vi "Test_sqlite.vi"() -> ()   [LabVIEW 2020]
uses:
  <vilib>/Viviota/shared/ORM.lvlibp/TypeMap/TypeMap.lvclass
  DbConnections/SqliteConnection/DBC.lvclass
  C:/Program Files/National Instruments/LabVIEW 2020/vi.lib/Viviota/shared/ORM.lvlibp/DbConnection/DbConnection.lvclass
  <vilib>/Viviota/shared/ORM_ADONet.lvlibp/ADOMapper/ADOMapper.lvclass
  C:/Program Files/National Instruments/LabVIEW 2020/vi.lib/Viviota/shared/ORM.lvlibp/SqlMapper/SqlMapper.lvclass
  <vilib>/Viviota/shared/ORM_lib.lvlibp/ObjectRow/ObjectLUT.lvclass
  <vilib>/numeric/Random Number (Range) I64.vi
  <vilib>/numeric/Random Number (Range) DBL.vi
  f3693442-7653-4e44-a421-498bef5f0c13.vi
  <vilib>/Analysis/baseanly.llb/Mean (DBL).vi
  <vilib>/numeric/sub_Random U32.vi
  <vilib>/JDP Science/JSONtext/Variant to JSON Text.vi
  <vilib>/Viviota/shared/ORM_lib.lvlibp/ObjectRow/Write LUT.vi
  <vilib>/Viviota/shared/ORM.lvlibp/DbConnection/Write SupportTX.vi
  <vilib>/Viviota/shared/ORM.lvlibp/SqlMapper/Write DbConnection.vi
  <vilib>/Viviota/shared/ORM.lvlibp/TypeMap/Write Table Name.vi
  <vilib>/Viviota/shared/ORM.lvlibp/TypeMap/Write Autokey.vi
  <vilib>/Viviota/shared/ORM.lvlibp/TypeMap/Write ExcludeIDFromQueryParam.vi
  <vilib>/Viviota/shared/ORM_lib.lvlibp/ObjectRow/Read LUT.vi
  <vilib>/JDP Science/JSONtext/LVClass Serializer/JSONtext LVClass Serializer.lvclass
  <vilib>/Analysis/NI_AALBase.lvlib
panel:
  out "error out":errorcluster
  out "mean 3":dbl format="%0.6f"
  out "mean 2":dbl format="%0.6f"
  out "mean":dbl format="%0.6f"
  out "x-y":dbl[](array[numeric])
  out "Array 2":dbl[](array[numeric])
  out "Array":dbl[](array[numeric])
  out "LUT 2":variant[](array[variant])
  out "LUT":variant[](array[variant])
  out "id":i32[](array[numeric])
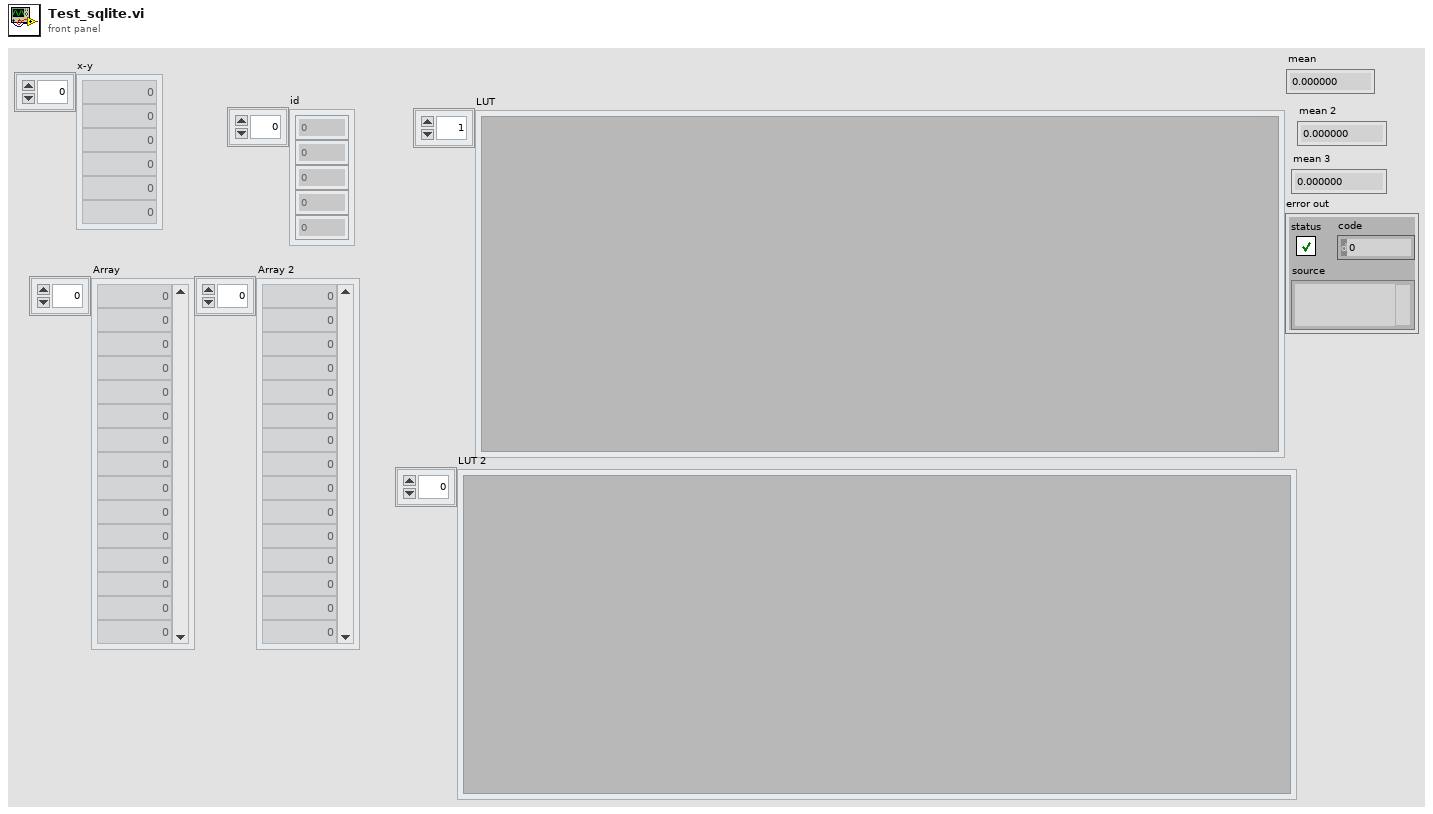
[diagram p1: front panel]
types:
  T1 = cluster{"Text":string, "Integer":i32, "dbl":dbl, "timestamp":timestamp}
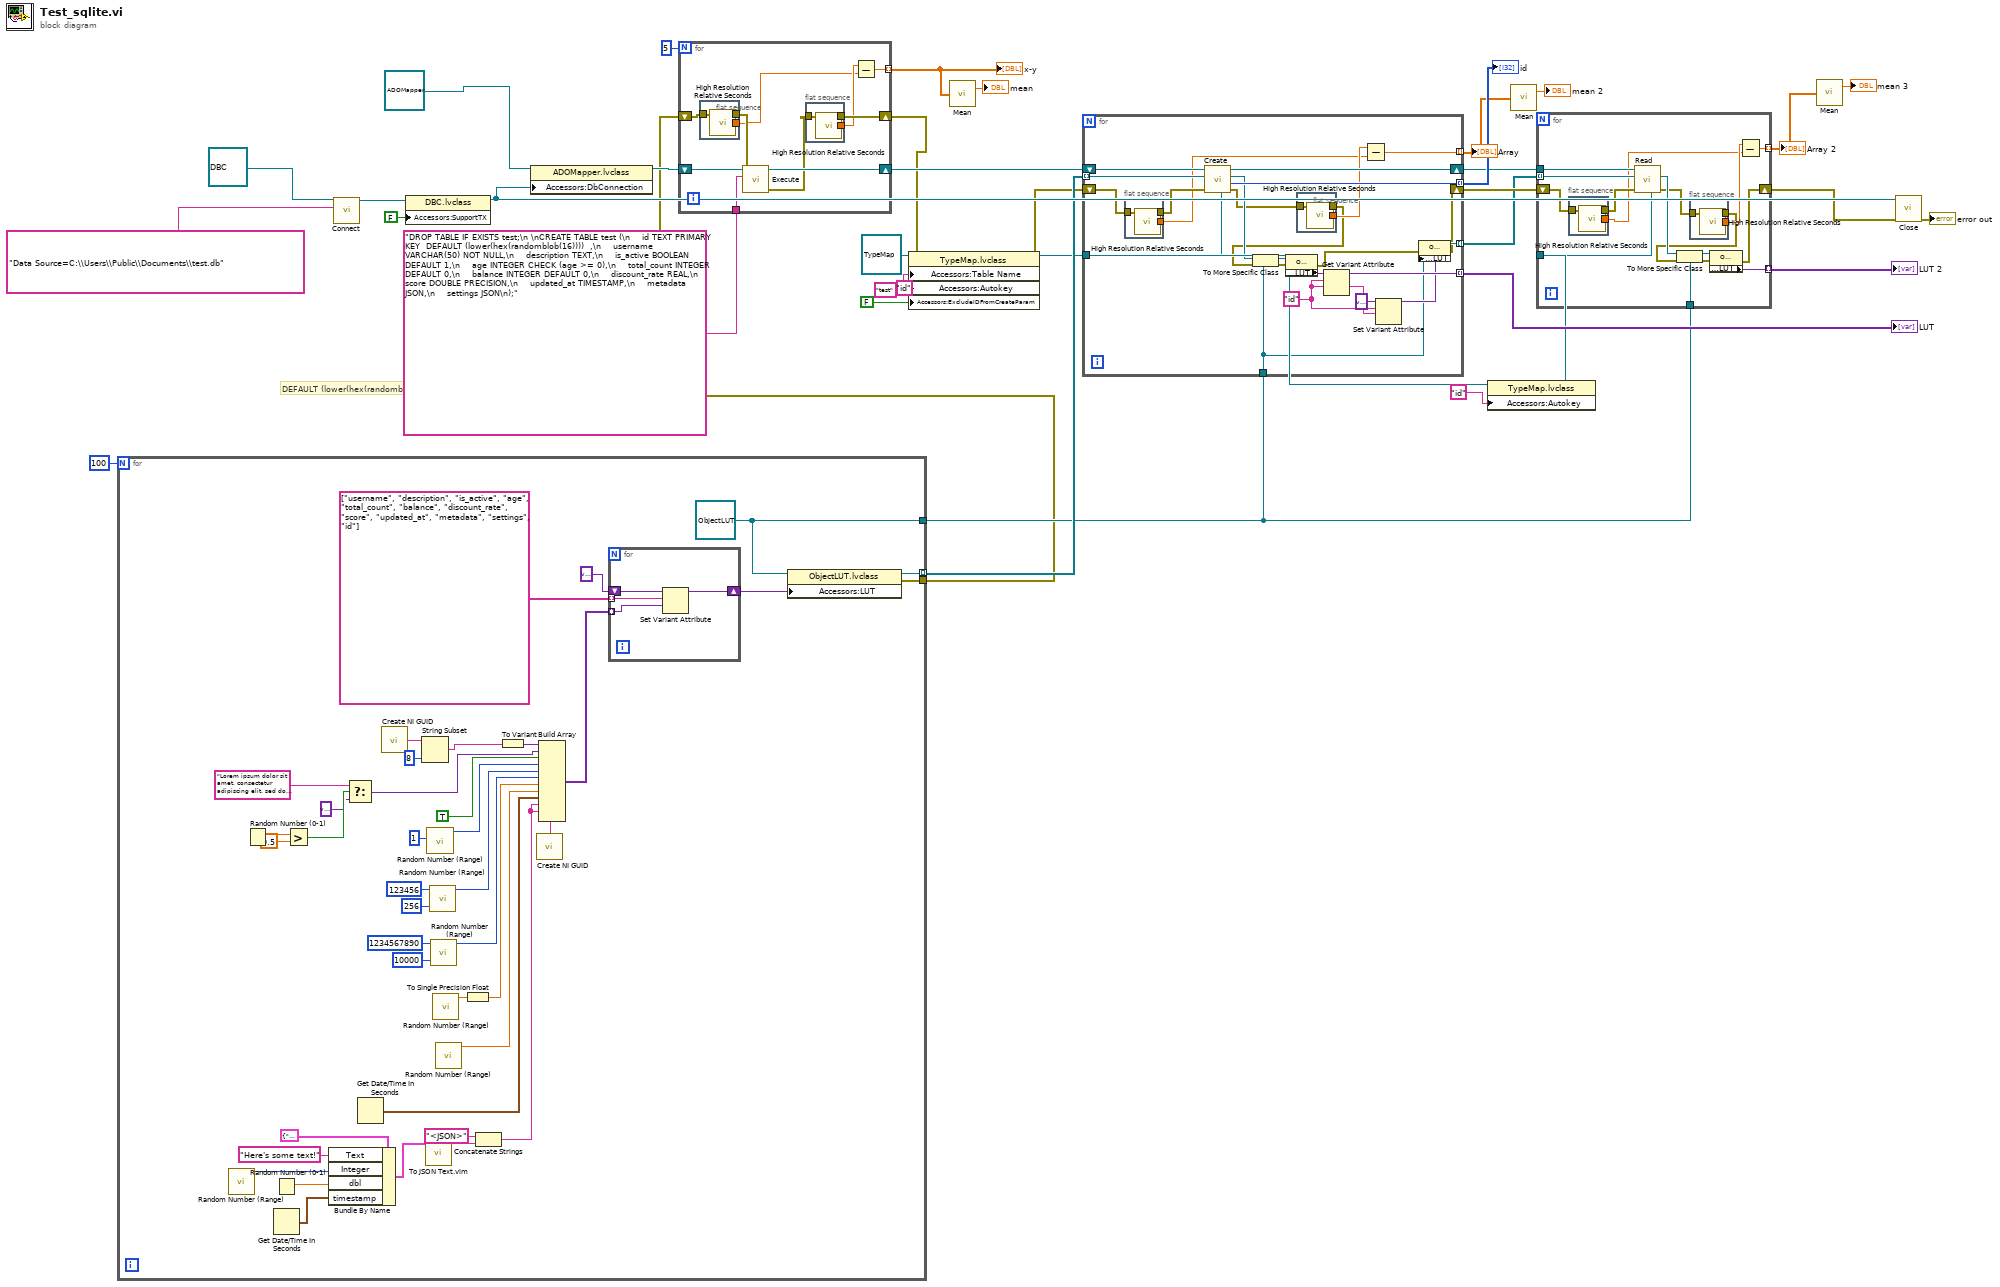
[diagram p0: block diagram]
diagram:
  # "DEFAULT (lower(hex(randomblob(16))))"
  n1 = for {
    N: 100 -> [_]
    tunnel: [w47] -> w31 mode=indexing
    tunnel: [w46] -> w21
    tunnel: [w41] -> w17
    w46 = refnum<class "ObjectLUT.lvclass"> refnum ("ORM_lib.lvlibp:ObjectLUT.lvclass")
    n2 = call-poly <vilib>:"Random Number (Range).vi"() -> ("number"=w54:i64)  [unwired: 11 in]
    n3 = Random Number (0-1)() -> (number: 0 to 1=w62:dbl)
    n4 = Random Number (0-1)() -> (number: 0 to 1=w55:dbl)
    n5 = Get Date/Time In Seconds() -> (seconds since 1Jan1904=w56:timestamp)
    n6 = Greater?(x=w62, y=0.5) -> (0:w60:bool)
    n7 = Bundle By Name(cluster=T1 {"Text"="This is a test", "Integer"=0, "dbl"=0.0, "timestamp"=timestamp(0 s since 1904-01-01)}, "Text"="Here's some text!", "Integer"=w54, "dbl"=w55, "timestamp"=w56) -> (w52:T1)
    n8 = Select(t="Lorem ipsum dolor sit amet, consectetur adipiscing elit, sed do eiusmod tempor incididunt ut labore et dolore magna aliqua", s=w60, f=variant) -> (s? t:f=w38:variant)
    n9 = Get Date/Time In Seconds() -> (seconds since 1Jan1904=w53:timestamp)
    n10 = call <vilib>:"Create NI GUID.vi"() -> ("NI GUID"=w77:string)
    n11 = String Subset(string=w77, length (rest)=8 ("length (rest)")) -> (substring=w72:string)  [unwired: 1 in]
    n12 = call "To JSON Text.vim"("Anything"=w52) -> ("<JSON>"=w45:string)  [unwired: 9 in, 1 out]
    n13 = call-poly <vilib>:"Random Number (Range).vi"("lower bound (-100)"=i64 1) -> ("number"=w69:i64)  [unwired: 10 in]
    n14 = call-poly <vilib>:"Random Number (Range).vi"("lower bound (-100)"=i64 256, "upper bound (100)"=i64 123456) -> ("number"=w68:i64)  [unwired: 9 in]
    n15 = call-poly <vilib>:"Random Number (Range).vi"("lower bound (-100)"=i64 10000, "upper bound (100)"=i64 1234567890) -> ("number"=w67:i64)  [unwired: 9 in]
    n16 = call-poly <vilib>:"Random Number (Range).vi"() -> ("number"=w65:dbl)  [unwired: 11 in]
    n17 = call-poly <vilib>:"Random Number (Range).vi"() -> ("number"=w63:dbl)  [unwired: 11 in]
    n18 = To Single Precision Float(number=w65) -> (single precision float=w64:sgl)
    n19 = Concatenate Strings("<JSON>" ("string"), w45) -> (w44:string)
    n20 = To Variant(anything=w72) -> (Variant=w71:variant)
    n21 = call <vilib>:"Create NI GUID.vi"() -> ("NI GUID"=w39:string)
    n22 = Build Array(w71, w38, TRUE, w69, w68, w67, w64, w63, w53, w44, w44, w39) -> (w50:variant[])
    n23 = for {
      tunnel: string[] ["username", "description", "is_active", "age", "total_count", "balance", "discount_rate", "score", "updated_at", "metadata", "settings", "id"] -> [w81] mode=indexing
      tunnel: w50 -> [w80] mode=indexing
      shift-right: [w79] -> w48
      shift-left: variant -> [w78]
      n24 = Set Variant Attribute(Variant=w78, name=w81, value=w80) -> (Variant out=w79:variant)  [unwired: 1 in, 2 out]
    }
    n25 = property class="ObjectLUT.lvclass"(reference=w46, "Accessors:LUT"=w48) -> (reference out=w47:refnum<class "ObjectLUT.lvclass">, error out=w41:errorcluster)  [unwired: 1 in]
  }
  n26 = call-dynamic "Connect.vi"("Connection String"="Data Source=C:\\Users\\Public\\Documents\\test.db", "SqliteConnection in"=refnum<class "DBC.lvclass"> refnum ("ORM_DBC_Sqlite.lvlib:DBC.lvclass")) -> ("SqliteConnection out"=w36:refnum<class "DBC.lvclass">)  [unwired: 8 in, 1 out]
  n27 = property class="DBC.lvclass"(reference=w36, "Accessors:SupportTX"=FALSE ("SupportTX")) -> (reference out=w32:refnum<class "DBC.lvclass">)  [unwired: 1 in, 1 out]
  n28 = property class="ADOMapper.lvclass"(reference=refnum<class "ADOMapper.lvclass"> refnum ("ORM_ADONet.lvlibp:ADOMapper.lvclass"), "Accessors:DbConnection"=w32) -> (reference out=w34:refnum<class "ADOMapper.lvclass">)  [unwired: 1 in, 1 out]
  n29 = for {
    N: 5 -> [_]
    tunnel: "DROP TABLE IF EXISTS test;\n \nCREATE TABLE test (\n    id TEXT PRIMARY KEY  DEFAULT (lower(hex(randomblob(16))))  ,\n    username VARCHAR(50) NOT NULL,\n    description TEXT,\n    is_active BOOLEAN DEFAULT 1,\n    age INTEGER CHECK (age >= 0),\n    total_count INTEGER DEFAULT 0,\n    balance INTEGER DEFAULT 0,\n    discount_rate REAL,\n    score DOUBLE PRECISION,\n    updated_at TIMESTAMP,\n    metadata JSON,\n    settings JSON\n);" ("sql") -> [w90]
    tunnel: [w82] -> w14 mode=indexing
    shift-right: [w89] -> w23
    shift-left: w34 -> [w91]
    shift-right: [w85] -> w16
    shift-left: w17 -> [w88]
    n30 = flat-sequence {
      tunnel: [w95] -> w83
      tunnel: w88 -> [w94]
      tunnel: [w94] -> w87
      frame #0 {
        n31 = call <vilib>:"High Resolution Relative Seconds.vi"() -> ("relative seconds"=w95:dbl)
      }
    }
    n32 = call-dynamic "Execute.vi"("error in (no error)"=w87, "sql"=w90, "ADOMapper in"=w91) -> ("error out"=w86:errorcluster, "ADOMapper out"=w89:refnum<class "ADOMapper.lvclass">)  [unwired: 6 in, 1 out]
    n33 = flat-sequence {
      tunnel: [w93] -> w84
      tunnel: w86 -> [w92]
      tunnel: [w92] -> w85
      frame #0 {
        n34 = call <vilib>:"High Resolution Relative Seconds.vi"() -> ("relative seconds"=w93:dbl)
      }
    }
    n35 = Subtract(x=w84, y=w83) -> (x-y=w82:dbl)
  }
  "x-y" <- w14
  n36 = property class="TypeMap.lvclass"(reference=refnum<class "TypeMap.lvclass"> refnum ("TypeMap in"), error in=w16, "Accessors:Table Name"="test" ("Table Name"), "Accessors:Autokey"="id" ("Autokey"), "Accessors:ExcludeIDFromCreateParam"=FALSE ("ExcludeIDFromCreateParam")) -> (reference out=w22:refnum<class "TypeMap.lvclass">, error out=w8:errorcluster)
  n37 = call-poly <vilib>:"Mean.vi"("X"=w14) -> ("mean"=→"mean":dbl)  [unwired: 1 out]
  n38 = for {
    tunnel: w31 -> [w119] mode=indexing
    tunnel: w22 -> [w118]
    tunnel: [w117] -> w28 mode=indexing
    tunnel: w21 -> [w107]
    tunnel: [w112] -> w27 mode=indexing
    shift-right: [w96] -> w25
    shift-left: w8 -> [w105]
    tunnel: [w106] -> w24 mode=indexing
    shift-right: [w102] -> w18
    shift-left: w23 -> [w120]
    tunnel: [w99] -> w10 mode=indexing
    w110 = "id" ("name")
    n39 = flat-sequence {
      tunnel: [w124] -> w100
      tunnel: w105 -> [w123]
      tunnel: [w123] -> w104
      frame #0 {
        n40 = call <vilib>:"High Resolution Relative Seconds.vi"() -> ("relative seconds"=w124:dbl)
      }
    }
    n41 = call-dynamic "Create.vi"("TypeMap in"=w118, "error in (no error)"=w104, "object in"=w119, "SqlMapper in"=w120) -> ("error out"=w103:errorcluster, "id"=w117:i32, "object out"=w116:refnum<class>, "SqlMapper out"=w102:refnum<class "SqlMapper.lvclass">)  [unwired: 4 in]
    n42 = To More Specific Class(target class=w107, reference=w116, error in=w98) -> (specific class reference=w114:refnum<class "ObjectLUT.lvclass">, error out=w115:errorcluster)
    n43 = property class="ObjectLUT.lvclass"(reference=w114, error in=w115) -> (error out=w97:errorcluster, "Accessors:LUT"=w113:variant)  [unwired: 1 out]
    n44 = flat-sequence {
      tunnel: [w122] -> w101
      tunnel: w103 -> [w121]
      tunnel: [w121] -> w98
      frame #0 {
        n45 = call <vilib>:"High Resolution Relative Seconds.vi"() -> ("relative seconds"=w122:dbl)
      }
    }
    n46 = Get Variant Attribute(Variant=w113, name=w110, default value (empty Variant)=w110) -> (duplicate Variant=w112:variant, value=w109:string)  [unwired: 1 in, 2 out]
    n47 = Subtract(x=w101, y=w100) -> (x-y=w99:dbl)
    n48 = Set Variant Attribute(Variant=variant ("variant"), name=w110, value=w109) -> (Variant out=w108:variant)  [unwired: 1 in, 2 out]
    n49 = property class="ObjectLUT.lvclass"(reference=w107, error in=w97, "Accessors:LUT"=w108) -> (reference out=w106:refnum<class "ObjectLUT.lvclass">, error out=w96:errorcluster)
  }
  "id" <- w28
  "LUT" <- w27
  "Array" <- w10
  n50 = property class="TypeMap.lvclass"(reference=w22, "Accessors:Autokey"="id" ("Autokey")) -> (reference out=w6:refnum<class "TypeMap.lvclass">)  [unwired: 1 in, 1 out]
  n51 = call-poly <vilib>:"Mean.vi"("X"=w10) -> ("mean"=→"mean 2":dbl)  [unwired: 1 out]
  n52 = for {
    tunnel: w24 -> [w140] mode=indexing
    tunnel: w18 -> [w139]
    tunnel: w6 -> [w138]
    tunnel: w21 -> [w134]
    tunnel: [w133] -> w20 mode=indexing
    shift-right: [w125] -> w19
    shift-left: w25 -> [w132]
    tunnel: [w127] -> w9 mode=indexing
    n53 = flat-sequence {
      tunnel: [w144] -> w128
      tunnel: w132 -> [w143]
      tunnel: [w143] -> w131
      frame #0 {
        n54 = call <vilib>:"High Resolution Relative Seconds.vi"() -> ("relative seconds"=w144:dbl)
      }
    }
    n55 = call-dynamic "Read.vi"("TypeMap in"=w138, "error in (no error)"=w131, "object in"=w140, "SqlMapper in"=w139) -> ("error out"=w130:errorcluster, "Value"=w135:refnum<class>)  [unwired: 4 in, 2 out]
    n56 = To More Specific Class(target class=w134, reference=w135, error in=w126) -> (specific class reference=w137:refnum<class "ObjectLUT.lvclass">, error out=w136:errorcluster)
    n57 = flat-sequence {
      tunnel: [w142] -> w129
      tunnel: w130 -> [w141]
      tunnel: [w141] -> w126
      frame #0 {
        n58 = call <vilib>:"High Resolution Relative Seconds.vi"() -> ("relative seconds"=w142:dbl)
      }
    }
    n59 = property class="ObjectLUT.lvclass"(reference=w137, error in=w136) -> (error out=w125:errorcluster, "Accessors:LUT"=w133:variant)  [unwired: 1 out]
    n60 = Subtract(x=w129, y=w128) -> (x-y=w127:dbl)
  }
  "LUT 2" <- w20
  "Array 2" <- w9
  n61 = call-poly <vilib>:"Mean.vi"("X"=w9) -> ("mean"=→"mean 3":dbl)  [unwired: 1 out]
  n62 = call-dynamic "Close.vi"("error in (no error)"=w19, "dbcDotNet in"=w32) -> ("error out"=→"error out":errorcluster)  [unwired: 9 in]
